vi "Untitled 4.vi"() -> ()   [LabVIEW 2018]
panel:
  in  "Numeric":dbl
  out "Meter":dbl(knob) scale=0.0..100.0
  out "Slide":dbl(slide) scale=0.0..10.0
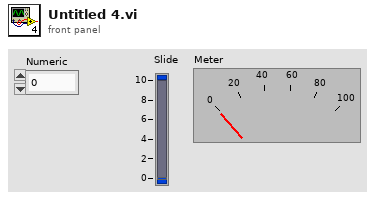
[diagram p1: front panel]
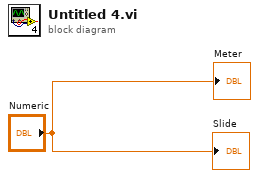
[diagram p0: block diagram]
diagram:
  "Slide" <- "Numeric"
  "Meter" <- "Numeric"
